vi "RDC-filter_box.vi"(7 "Lower Cut-Off":dbl=30000.0 format="%#_13g", 11 "input cluster":T1) -> (3 "output cluster":T1)   [LabVIEW 2020, in "RDC-Reflection_Data_Computation.lvlib"]
doc: "Filters the data of a Common Format cluster with a lower cut-off and returns the filtered cluster."
uses:
  RDC-Reflection_Data_Computation.lvlib
  Reflector/RFH-common_data_format.ctl
  Reflector/RFH-Reflection_File_Handler.lvlib
panel:
  out "Waveform Graph 6":dbl[][](graph)
  out "Numeric":i32
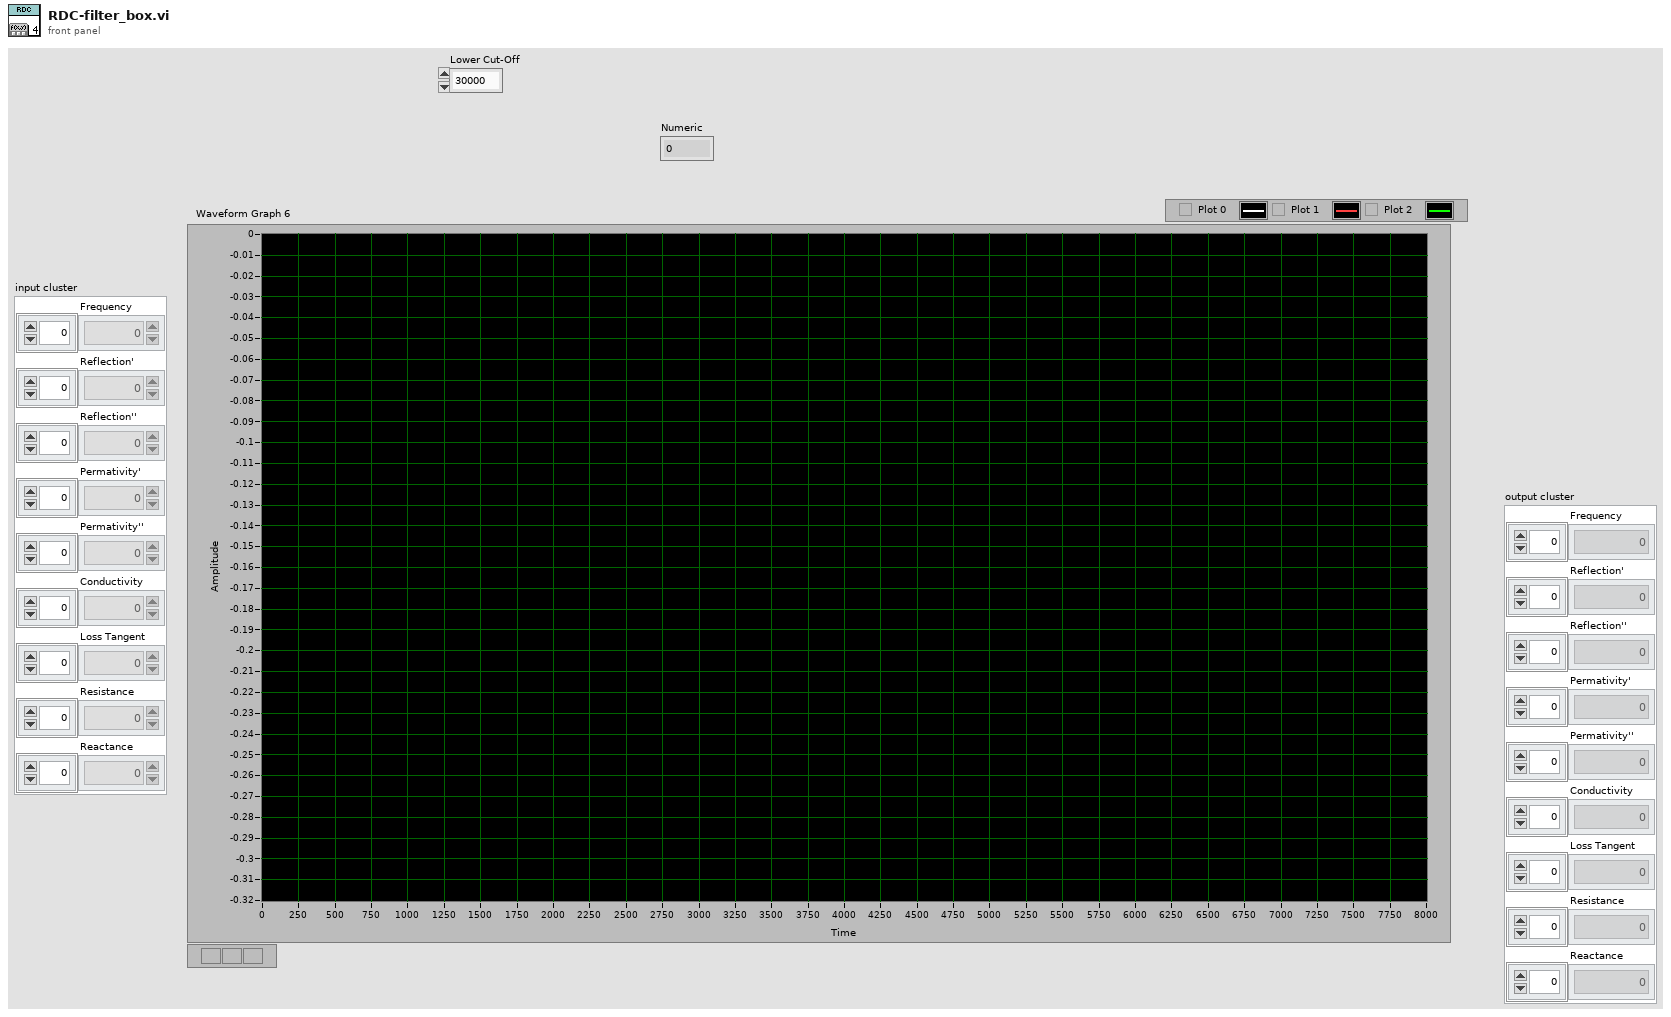
[diagram p1: front panel]
types:
  T1 = typedef "RFH-Reflection_File_Handler.lvlib/RFH-common_data_format.ctl" = cluster{"Frequency":dbl[], "Reflection'":dbl[], "Reflection''":dbl[], "Permativity'":dbl[], "Permativity''":dbl[], "Conductivity":dbl[], "Loss Tangent":dbl[], "Resistance":dbl[], "Reactance":dbl[]}
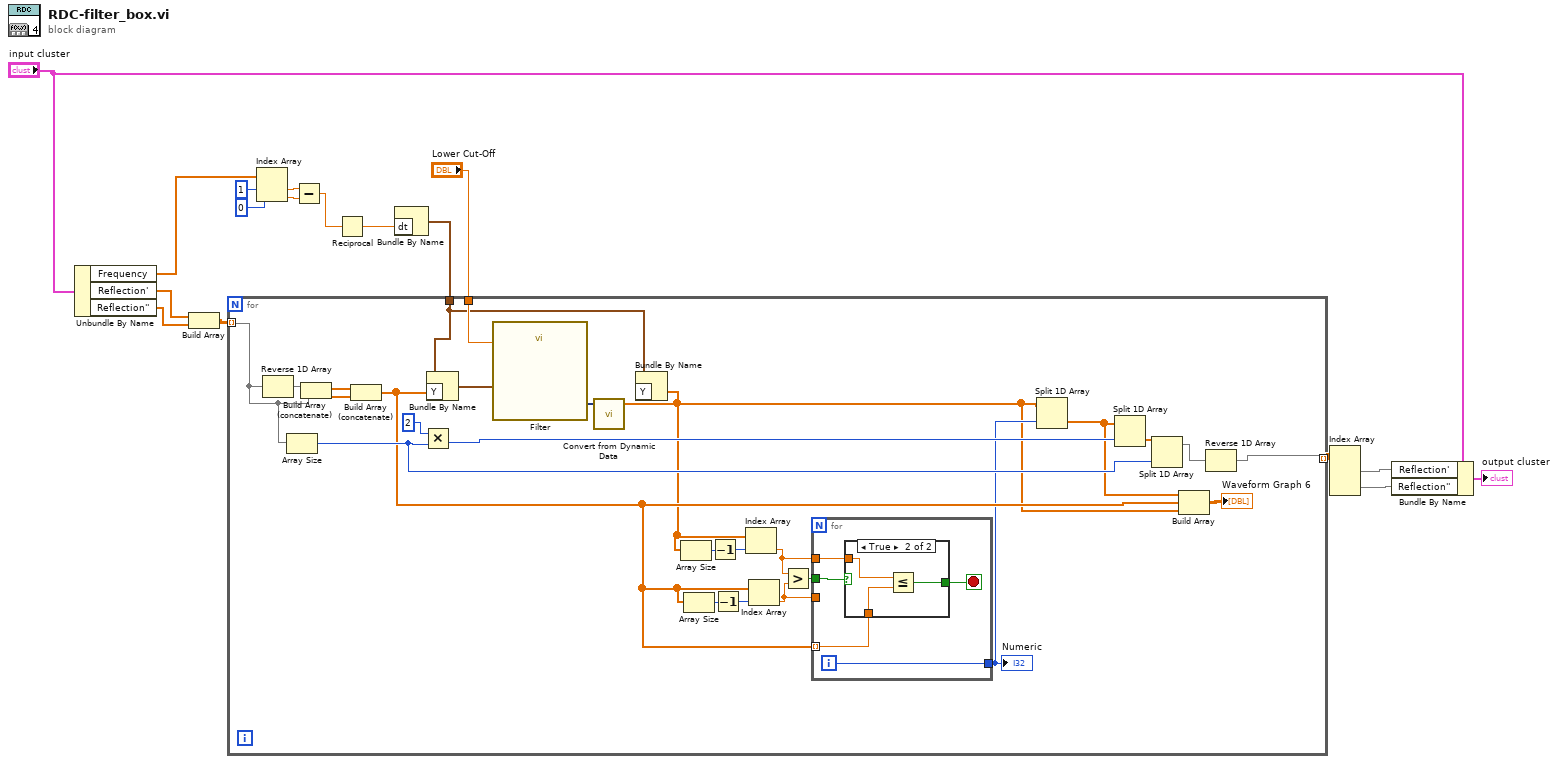
[diagram p0: block diagram]
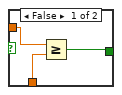
[diagram p2: hidden frame]
diagram:
  n1 = Unbundle By Name("input cluster") -> ("Frequency"=w16:dbl[], "Reflection'"=w9:dbl[], "Reflection''"=w8:dbl[])
  n2 = Build Array(w9, w8) -> (w7:dbl[][])
  n3 = Index Array(array=w16, index #1=1 ("index"), index #2=0 ("index")) -> (element #1=w13:dbl, element #2=w12:dbl)
  n4 = Subtract(x=w13, y=w12) -> (x-y=w11:dbl)
  n5 = Reciprocal(x=w11) -> (1/x=w1:dbl)
  n6 = Bundle By Name("dt"=w1) -> (w10:waveform(dbl))  [unwired: 1 in]
  n7 = for {
    tunnel: "Lower Cut-Off" -> [w41]
    tunnel: w10 -> [w29]
    tunnel: w7 -> [w33] mode=indexing
    tunnel: [w32] -> w5 mode=indexing
    n8 = Reverse 1D Array(array=w33) -> (reversed array=w42:dbl[])
    n9 = Array Size(array=w33) -> (size(s)=w30:i32)
    n10 = Build Array (concatenate)(w42, w33) -> (w39:dbl[])
    n11 = Build Array (concatenate)(w39, w39) -> (w24:dbl[])
    n12 = Multiply(x=2, y=w30) -> (x*y=w31:i32)
    n13 = Bundle By Name(cluster=w29, "Y"=w24) -> (w34:waveform(dbl))
    n14 = call "Filter"("Lower Cut-Off"=w41, "Signal"=w34) -> ("Filtered Signal"=w35:dynamicdata)  [unwired: 8 in, 1 out]
    n15 = call "Convert from Dynamic Data"("Dynamic Data Type"=w35) -> ("Array"=w18:dbl[])  [unwired: 3 in]
    n16 = Bundle By Name(cluster=w29, "Y"=w18) -> ()  [unwired: 1 out]
    n17 = Array Size(array=w18) -> (size(s)=w28:i32)
    n18 = Array Size(array=w24) -> (size(s)=w25:i32)
    n19 = Decrement(x=w28) -> (x-1=w27:i32)
    n20 = Decrement(x=w25) -> (x-1=w26:i32)
    n21 = Index Array(array=w18, index=w27) -> (element=w22:dbl)
    n22 = Index Array(array=w24, index=w26) -> (element=w21:dbl)
    n23 = Greater?(x=w22, y=w21) -> (0:w23:bool)
    n24 = for {
      tunnel: w24 -> [w44] mode=indexing
      tunnel: w23 -> [w47]
      tunnel: w22 -> [w46]
      tunnel: w21 -> [_]
      tunnel: [w43] -> w20
      i -> [w43]
      stop <- w45 stop-if-true
      n25 = case shown="True" w47 {
        tunnel: w46 -> [w50 w53]
        tunnel: [w49 w52] -> w45
        tunnel: w44 -> [w48 w51]
        frame False {
          n26 = Greater Or Equal?(x=w50, y=w48) -> (x >= y?=w49:bool)
        }
        frame True {
          n27 = Less Or Equal?(x=w53, y=w51) -> (x <= y?=w52:bool)
        }
      }
    }
    "Numeric" <- w20
    n28 = Split 1D Array(array=w18, index=w20) -> (second subarray=w19:dbl[])  [unwired: 1 out]
    n29 = Split 1D Array(array=w19, index=w31) -> (second subarray=w38:dbl[])  [unwired: 1 out]
    n30 = Split 1D Array(array=w38, index=w30) -> (first subarray=w37:dbl[])  [unwired: 1 out]
    n31 = Build Array(w19, w24, w18) -> (→"Waveform Graph 6":dbl[][])
    n32 = Reverse 1D Array(array=w37) -> (reversed array=w32:dbl[])
  }
  n33 = Index Array(array=w5) -> (element #1=w4:dbl[], element #2=w3:dbl[])  [unwired: 4 in]
  n34 = Bundle By Name(cluster="input cluster", "Reflection'"=w4, "Reflection''"=w3) -> (→"output cluster":T1)
